vi "Script Rich to Flat Oneof Conversion.vi"(5 "element metadata":T1={"Field Name"="", "Embedded Message Name"="", "Protobuf Index"=1, "MessageElementType"=enum."StringValue", "Repeated"=FALSE, "Is in Oneof"=FALSE, "Oneof Container Name"=""}, 7 "library in":refnum<vi>, 8 "error in (no error)":errorcluster, 9 "unbundler":refnum<vi>, 10 "bundler":refnum<vi>, 11 "vi in":refnum<vi>) -> (0 "error out":errorcluster, 3 "vi out":refnum<vi>)   [LabVIEW 2019, in "gRPC Template Creation Utility.lvlib"]
uses:
  gRPC Template Creation Utility.lvlib
  TypeDefs/Message Element Metadata (Scripting).ctl
  TypeDefs/Message Element Type.ctl
  OneOf Constants/OneOfConstantsEnum.ctl
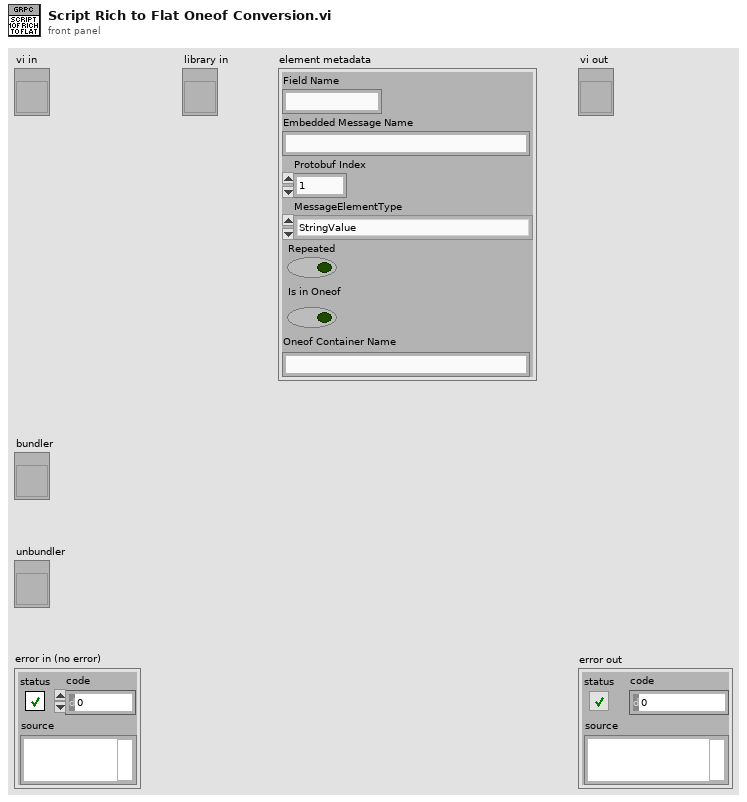
[diagram p1: front panel]
types:
  T1 = typedef "gRPC Template Creation Utility.lvlib/Message Element Metadata (Scripting).ctl" = cluster{"Field Name":string, "Embedded Message Name":string, "Protobuf Index":i32, "MessageElementType":T2, "Repeated":bool, "Is in Oneof":bool, "Oneof Container Name":string}
  T2 = typedef "gRPC Template Creation Utility.lvlib/Message Element Type.ctl" = enum32{"Int32Value", "FloatValue", "DoubleValue", "BoolValue", "StringValue", "MessageValue", "Int64Value", "UInt32Value", "UInt64Value", "EnumValue", "Bytes", "Fixed64", "Fixed32", "SFixed64", "SFixed32", "SInt64", "SInt32"}
  T3 = typedef "gRPC Template Creation Utility.lvlib/OneOfConstantsEnum.ctl" = enum16{"FlatToRichVIPrefix", "RichToFlatVIPrefix", "FlatTypeDefSuffix"}
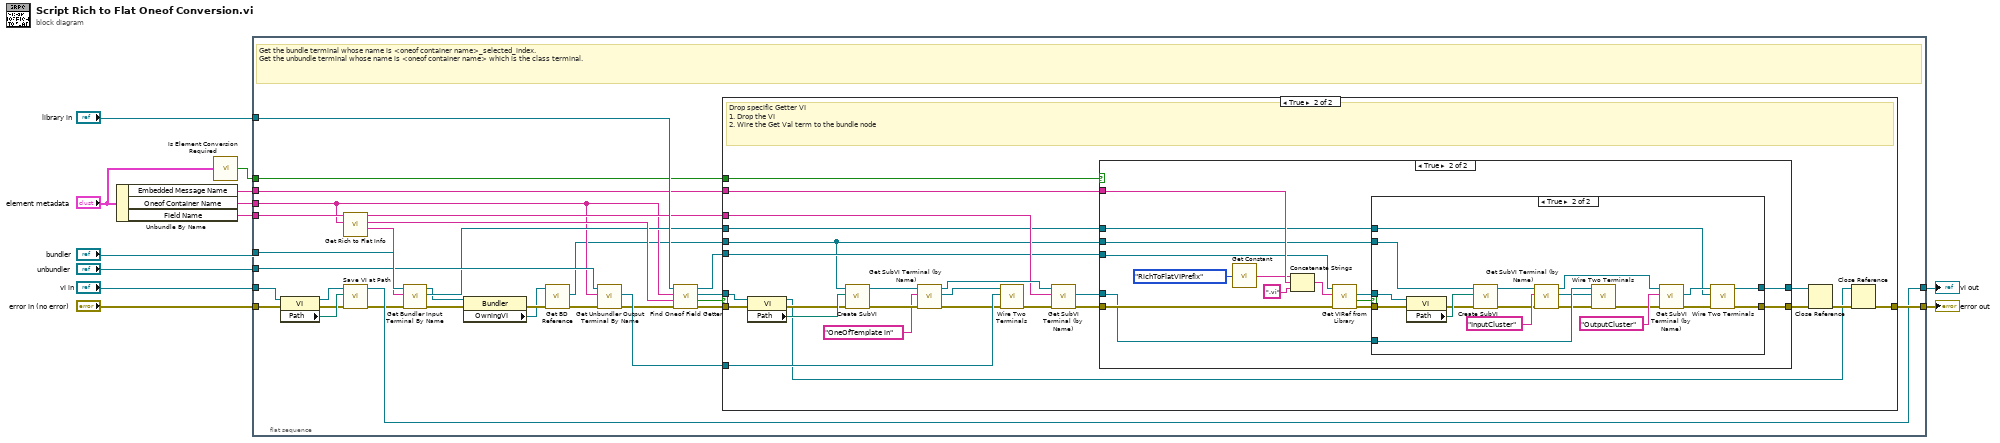
[diagram p0: block diagram]
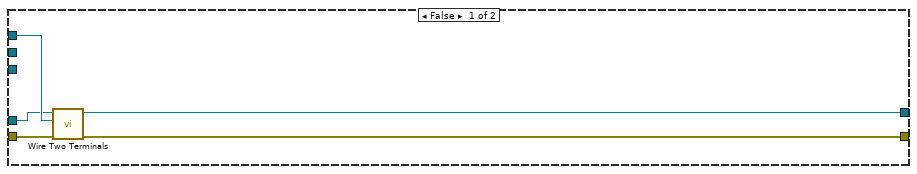
[diagram p3: hidden frame]
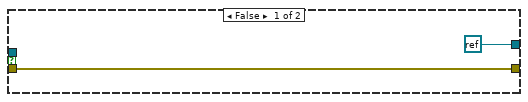
[diagram p4: hidden frame]
diagram:
  n1 = Unbundle By Name("element metadata") -> ("Embedded Message Name"=w7:string, "Oneof Container Name"=w9:string, "Field Name"=w8:string)
  n2 = call "Is Element Conversion Required.vi"("element metadata"="element metadata") -> ("conversion required"=w2:bool)
  n3 = flat-sequence {
    tunnel: w9 -> [w22]
    tunnel: w8 -> [w25]
    tunnel: "error in (no error)" -> [w18]
    tunnel: [w35] -> w11
    tunnel: "bundler" -> [w43]
    tunnel: "unbundler" -> [w42]
    tunnel: "vi in" -> [w41]
    tunnel: "library in" -> [w34]
    tunnel: [w31] -> w12
    tunnel: w2 -> [w21]
    tunnel: w7 -> [w20]
    frame #0 {
      # "Get the bundle terminal whose name is <oneof container name>_selected_index.\nGet the unbundle terminal whose name is <oneof container name> which is the class terminal."
      n4 = property class="VI"(reference=w41, error in=w18) -> (reference out=w33:refnum<vi>, error out=w30:errorcluster, "Path"=w32:path)
      n5 = call "Get Rich to Flat Info.vi"("oneof container name"=w22, "field name"=w25) -> ("bundler terminal name"=w23:string, "getter vi name"=w38:string, "get value terminal name"=w24:string)  [unwired: 7 in]
      n6 = call "Save VI at Path.vi"("error in (no error)"=w30, "Path"=w32, "VI in"=w33) -> ("error out"=w17:errorcluster, "VI out"=w31:refnum<vi>)  [unwired: 6 in, 1 out]
      n7 = call "Get Bundler Input Terminal By Name.vi"("error in (no error)"=w17, "Terminal name"=w23, "Bundler in"=w43) -> ("error out"=w16:errorcluster, "Terminal Refnum"=w29:refnum<vi>, "Bundler out"=w28:refnum<vi>)  [unwired: 5 in, 1 out]
      n8 = property class="Bundler"(reference=w28, error in=w16) -> (error out=w27:errorcluster, "OwningVI"=w26:refnum<vi>)  [unwired: 1 out]
      n9 = call "Get BD Reference.vi"("error in"=w27, "VI in"=w26) -> ("error out"=w15:errorcluster, "Block Diagram"=w13:refnum<vi>)  [unwired: 7 in, 1 out]
      n10 = call "Get Unbundler Output Terminal By Name.vi"("error in (no error)"=w15, "Terminal name"=w22, "Unbundler in"=w42) -> ("error out"=w14:errorcluster, "Terminal Refnum"=w37:refnum<vi>)  [unwired: 5 in, 2 out]
      n11 = call "Find Oneof Field Getter.vi"("error in (no error)"=w14, "getter vi name"=w38, "oneof container name"=w22, "library in"=w34) -> ("error out"=w36:errorcluster, "found?"=w39:bool, "getter vi"=w40:refnum<vi>, "library out"=w19:refnum<vi>)  [unwired: 4 in]
      n12 = case shown="True" w39 {
        tunnel: w40 -> [_ w69]
        tunnel: w37 -> [_ w65]
        tunnel: w36 -> [w44 w61]
        tunnel: [w44 w58] -> w35
        tunnel: w29 -> [_ w50]
        tunnel: w13 -> [_ w45]
        tunnel: w24 -> [_ w54]
        tunnel: w21 -> [_ w53]
        tunnel: w20 -> [_ w52]
        tunnel: w19 -> [_ w46]
        frame False {
          # "TODO: Add error because we didn't find the getter VI"
        }
        frame True {
          # "Drop specific Getter VI\n1. Drop the VI\n2. Wire the Get Val term to the bundle node"
          n13 = property class="VI"(reference=w69, error in=w61) -> (reference out=w59:refnum<vi>, error out=w62:errorcluster, "Path"=w68:path)
          n14 = call "Create SubVI.vi"("error in (no error)"=w62, "Path"=w68, "Diagram in"=w45) -> ("error out"=w63:errorcluster, "subVI refnum"=w67:refnum<vi>)  [unwired: 7 in]
          n15 = call "Get SubVI Terminal (by Name).vi"("error in (no error)"=w63, "Terminal name"="OneOfTemplate in", "SubVI in"=w67) -> ("error out"=w64:errorcluster, "SubVI Term ref"=w66:refnum<vi>, "SubVI out"=w56:refnum<vi>)  [unwired: 5 in, 1 out]
          n16 = call "Wire Two Terminals.vi"("error in (no error)"=w64, "Sink Terminal in"=w65, "Source Terminal"=w66) -> ("error out"=w55:errorcluster)  [unwired: 7 in, 1 out]
          n17 = call "Get SubVI Terminal (by Name).vi"("error in (no error)"=w55, "Terminal name"=w54, "SubVI in"=w56) -> ("error out"=w51:errorcluster, "SubVI Term ref"=w49:refnum<vi>)  [unwired: 5 in, 2 out]
          n18 = case shown="True" w53 {
            tunnel: w52 -> [_ w87]
            tunnel: w51 -> [w74 w85]
            tunnel: w50 -> [w73 w78]
            tunnel: w49 -> [w72 w79]
            tunnel: [w71 w80] -> w48
            tunnel: [w70 w77] -> w47
            tunnel: w46 -> [_ w86]
            tunnel: w45 -> [_ w82]
            frame False {
              n19 = call "Wire Two Terminals.vi"("error in (no error)"=w74, "Sink Terminal in"=w73, "Source Terminal"=w72) -> ("error out"=w71:errorcluster, "Source Terminal out"=w70:refnum<vi>)  [unwired: 7 in]
            }
            frame True {
              n20 = call "Get Constant.vi"("Selection"=OneOfConstantsEnum."RichToFlatVIPrefix") -> ("String"=w75:string)
              n21 = Concatenate Strings(w75, w87, ".vi" ("string")) -> (w88:string)
              n22 = call "Get VIRef from Library.vi"("error in (no error)"=w85, "item name"=w88, "library in"=w86) -> ("error out"=w83:errorcluster, "found"=w84:bool, "vi"=w81:refnum<vi>)  [unwired: 5 in, 1 out]
              n23 = case shown="True" w84 {
                tunnel: [w91 w96] -> w80
                tunnel: w83 -> [w91 w94]
                tunnel: w82 -> [_ w110]
                tunnel: w81 -> [_ w109]
                tunnel: w79 -> [_ w104]
                tunnel: w78 -> [_ w92]
                tunnel: [refnum<k0> refnum w95] -> w77
                frame False {
                }
                frame True {
                  n24 = property class="VI"(reference=w109, error in=w94) -> (error out=w93:errorcluster, "Path"=w108:path)  [unwired: 1 out]
                  n25 = call "Create SubVI.vi"("error in (no error)"=w93, "Path"=w108, "Diagram in"=w110) -> ("error out"=w105:errorcluster, "subVI refnum"=w107:refnum<vi>)  [unwired: 7 in]
                  n26 = call "Get SubVI Terminal (by Name).vi"("error in (no error)"=w105, "Terminal name"="InputCluster", "SubVI in"=w107) -> ("error out"=w102:errorcluster, "SubVI Term ref"=w103:refnum<vi>, "SubVI out"=w99:refnum<vi>)  [unwired: 5 in, 1 out]
                  n27 = call "Wire Two Terminals.vi"("error in (no error)"=w102, "Sink Terminal in"=w103, "Source Terminal"=w104) -> ("error out"=w100:errorcluster)  [unwired: 7 in, 1 out]
                  n28 = call "Get SubVI Terminal (by Name).vi"("error in (no error)"=w100, "Terminal name"="OutputCluster", "SubVI in"=w99) -> ("error out"=w97:errorcluster, "SubVI Term ref"=w98:refnum<vi>)  [unwired: 5 in, 2 out]
                  n29 = call "Wire Two Terminals.vi"("error in (no error)"=w97, "Sink Terminal in"=w92, "Source Terminal"=w98) -> ("error out"=w96:errorcluster, "Source Terminal out"=w95:refnum<vi>)  [unwired: 7 in]
                }
              }
            }
          }
          n30 = Close Reference(reference=w47, error in (no error)=w48) -> (error out=w60:errorcluster)
          n31 = Close Reference(reference=w59, error in (no error)=w60) -> (error out=w58:errorcluster)
        }
      }
    }
  }
  "error out" <- w11
  "vi out" <- w12
